vi "Get Status.vi"(8 "error in (no error)":errorcluster, 11 "AS7431 Light Spectrum in":refnum<class "AS7431 11 Ch Light Spectrum Sensor.lvclass">) -> (0 "error out":errorcluster, 2 "Data":string, 3 "AS7431 Light Spectrum out":refnum<class "AS7431 11 Ch Light Spectrum Sensor.lvclass">)   [LabVIEW 2020, in "CTI-Peripheral.lvlib" / "AS7431 11 Ch Light Spectrum Sensor.lvclass"]
uses:
  AS7431 11 Ch Light Spectrum Sensor.lvclass
  AS7431 11 Ch Light Spectrum Sensor.lvclass/AS7431 11 Ch Light Spectrum Sensor.ctl
  CTI/I2C Connection/I2C Connection.lvclass/I2C Connection.ctl
  CTI/Session/I2C Write Data.vi
  CTI/Session/I2C Read Data.vi
  CTI/I2C Connection/I2C Connection.lvclass
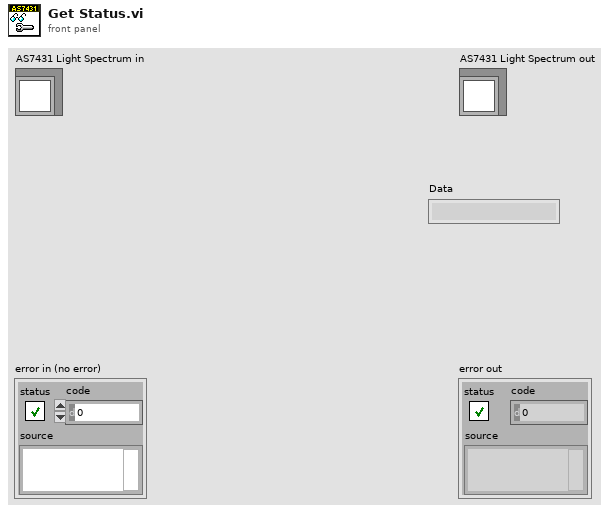
[diagram p1: front panel]
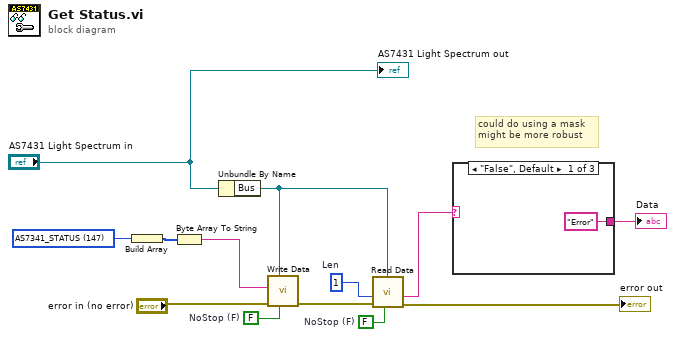
[diagram p0: block diagram]
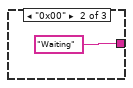
[diagram p2: hidden frame]
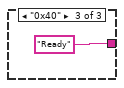
[diagram p3: hidden frame]
diagram:
  w5 = u16 147 items=["AS7341_I2CADDR_DEFAULT"=57, "AS7341_CHIP_ID"=9, "AS7341_WHOAMI"=146, "AS7341_CONFIG"=112, "AS7341_GPIO"=115, "AS7341_LED"=116, "AS7341_ENABLE"=128, "AS7341_ATIME"=129, "AS7341_SP_LOW_TH_L"=132, "AS7341_SP_LOW_TH_H"=133, "AS7341_SP_HIGH_TH_L"=134, "AS7341_SP_HIGH_TH_H"=135, "AS7341_STATUS"=147, "AS7341_ASTATUS_"=148, "AS7341_CH0_DATA_L"=149, "AS7341_CH0_DATA_H"=150, "AS7341_CH1_DATA_L"=151, "AS7341_CH1_DATA_H"=152, "AS7341_CH2_DATA_L"=153, "AS7341_CH2_DATA_H"=154, "AS7341_CH3_DATA_L"=155, "AS7341_CH3_DATA_H"=156, "AS7341_CH4_DATA_L"=157, "AS7341_CH4_DATA_H"=158, "AS7341_CH5_DATA_L"=159, "AS7341_CH5_DATA_H"=160, "AS7341_STATUS2"=163, "AS7341_STATUS3"=164, "AS7341_CFG0"=169, "AS7341_CFG1"=170, "AS7341_CFG6"=175, "AS7341_CFG9"=178, "AS7341_CFG12"=181, "AS7341_PERS"=189, "AS7341_GPIO2"=190, "AS7341_ASTEP_L"=202, "AS7341_ASTEP_H"=203, "AS7341_FD_TIME1"=216, "AS7341_FD_TIME2"=218, "AS7341_FD_STATUS"=219, "AS7341_INTENAB"=249, "AS7341_CONTROL"=250] ("Registers")
  w10 = FALSE  # NoStop (F)
  w11 = u8 1  # Len
  w12 = FALSE  # NoStop (F)
  # "could do using a mask\nmight be more robust"
  n1 = Build Array(w5) -> (w4:u16[])
  n2 = Byte Array To String(unsigned byte array=w4) -> (string=w3:string)
  n3 = Unbundle By Name("AS7431 Light Spectrum in") -> ("Bus"=w9:refnum<class "I2C Connection.lvclass">)
  n4 = call "Write Data.vi"("NoStop (F)"=w12, "I2C Connection"=w9, "error in (no error)"="error in (no error)", "Data"=w3) -> ("error out"=w8:errorcluster)  [unwired: 7 in]
  n5 = call "Read Data.vi"("NoStop (F)"=w10, "I2C Connection"=w9, "error in (no error)"=w8, "Len"=w11) -> ("error out"=→"error out":errorcluster, "Data"=w2:string)  [unwired: 6 in]
  n6 = case shown="\"False\", Default" w2 {
    tunnel: ["Error" ("Data") "Waiting" ("Data") "Ready" ("Data")] -> w1
    frame "False", Default {
    }
    frame "0x00" {
    }
    frame "0x40" {
    }
  }
  "Data" <- w1
  "AS7431 Light Spectrum out" <- "AS7431 Light Spectrum in"
